vi "UE_Capture_Acceptable.vi"(3 "buffer_ok":bool, 4 "feedback_valid":bool, 5 "samples_present":bool) -> (2 "acceptable":bool)   [LabVIEW 2026]
doc: "INTENT: Accept a completed capture only when samples exist, feedback is valid and buffer succeeded. INPUTS: samples_present (bool), feedback_valid (bool), buffer_ok (bool). OUTPUTS: acceptable (bool). DESIGN CONSTRAINT: Does not perform logging, average calculation or buffer management. REQUIREMENTS: SRS-F-008. No physical hardware side effects. Acceptance requires native LabVIEW compilation and behavioral testing."
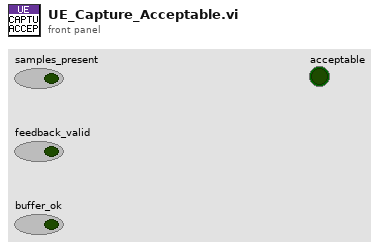
[diagram p1: front panel]
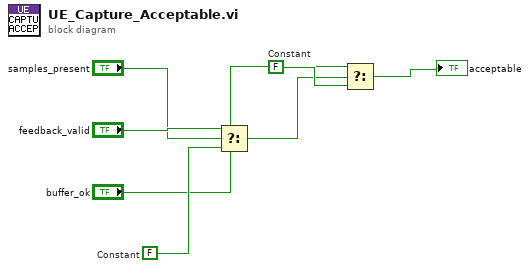
[diagram p0: block diagram]
diagram:
  w6 = FALSE  # Constant
  w4 = FALSE  # Constant
  n1 = Select(t="feedback_valid", s="samples_present", f=w4) -> (s? t:f=w5:bool)
  n2 = Select(t="buffer_ok", s=w5, f=w6) -> (s? t:f=→"acceptable":bool)
